vi "Read Reader.vi"(8 "error in (no error)":errorcluster, 11 "ADOResult in":refnum<class "ADOResult.lvclass">) -> (0 "error out":errorcluster, 2 "Reader":refnum<k39>, 3 "ADOResult out":refnum<class "ADOResult.lvclass">)   [LabVIEW 2026, in "ORM_ADONetCore.lvlib" / "ADOResult.lvclass"]
uses:
  ADOResult.lvclass
  C:/Program Files/dotnet/shared/Microsoft.NETCore.App/8.0.28/System.Data.Common.dll
  Program Files/dotnet/shared/Microsoft.NETCore.App/8.0.28/System.Data.Common.dll
  ADOResult.lvclass/ADOResult.ctl
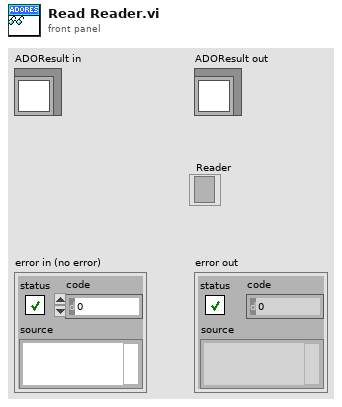
[diagram p1: front panel]
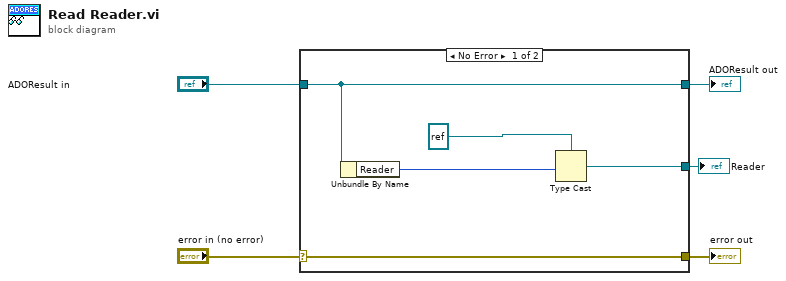
[diagram p0: block diagram]
diagram:
  n1 = case shown="No Error" "error in (no error)" {
    selector: "error in (no error)" -> [w10 w11]
    tunnel: [w10 w11] -> w4
    tunnel: [w9 w12] -> w2
    tunnel: "ADOResult in" -> [w9 w12]
    tunnel: [w7 _] -> w1
    frame No Error {
      n2 = Unbundle By Name(w9) -> ("Reader"=w8:u64)
      n3 = Type Cast(type=refnum<k39> refnum ("ExecuteReader"), x=w8) -> (*(type *) &x=w7:refnum<k39>)
    }
    frame Error {
    }
  }
  "error out" <- w4
  "ADOResult out" <- w2
  "Reader" <- w1
